vi "mupEval.vi"(8 "error in (no error)":errorcluster, 11 "hParser in":u64) -> (0 "error out":errorcluster, 2 "result":dbl, 3 "hParser out":u64)   [LabVIEW 2018, in "mupLib.lvlib"]
doc: "Evaluate the expression and return a single result.\n\nIf multiple expressions have been input, the last one in the list is evaluated.\n\nIf the variables are defined for bulk mode evaluation, only the first set (index 0) will be evaluiated."
uses:
  mupLib.lvlib
  <vilib>/Utility/error.llb/Error Cluster From Error Code.vi
  libmuparser-lv.dll
panel:
  # "Evaluate the expression and return a single result.\n\nIf multiple expressions have been input, the last one in the list is evaluated.\n\nIf the variables are defined for bulk mode evaluation, only the first set (index 0) will be evaluiated."
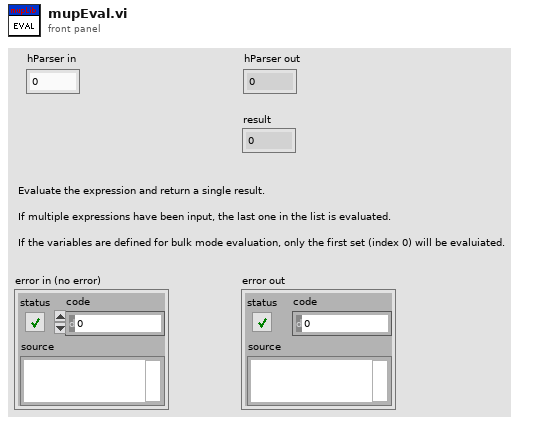
[diagram p1: front panel]
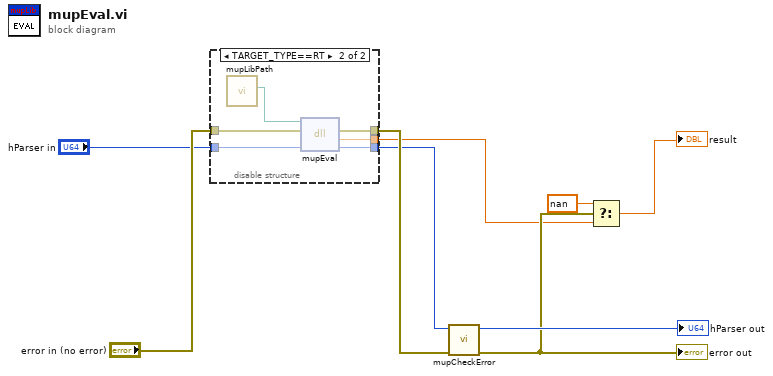
[diagram p0: block diagram]
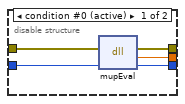
[diagram p2: hidden frame]
diagram:
  n1 = disable-structure shown="TARGET_TYPE==RT" {
    disable-tunnel: [w14 w20] -> w9
    disable-tunnel: "error in (no error)" -> [w13 w19]
    disable-tunnel: [w12 w18] -> w5
    disable-tunnel: "hParser in" -> [w11 w17]
    disable-tunnel: [w10 w16] -> w1
    frame condition #0 (active) {
      n2 = dll-call lib="C:/Users/leonidas/Documents/GitHub/LV-muParser/mupLib/libmuparser-lv.dll" fn="mupEval"(error in=w13, "hParser"=w11) -> (error out=w14:errorcluster, "return type"=w12:dbl, "hParser"=w10:u64)  [unwired: 2 in, 1 out]
    }
    frame condition #1 {
      n3 = call "mupLibPath.vi"() -> ("libmuparser path"=w15:path)  [unwired: 11 in]
      n4 = dll-call lib="C:/Users/leonidas/Documents/GitHub/LV-muParser/mupLib/libmuparser-lv.dll" fn="mupEval"(path in=w15, error in=w19, "hParser"=w17) -> (error out=w20:errorcluster, "return type"=w18:dbl, "hParser"=w16:u64)  [unwired: 1 in, 1 out]
    }
  }
  n5 = call "mupCheckError.vi"("error in (no error)"=w9, "hParser in"=w1) -> ("error out"=w6:errorcluster, "hParser out"=→"hParser out":u64)  [unwired: 8 in]
  "error out" <- w6
  n6 = Select(t=nan, s=w6, f=w5) -> (s? t:f=→"result":dbl)
